vi "Init Module.vi"(8 "error in":errorcluster, 10 "Close Master Reference (F)":bool, 11 "Cloneable Module Admin in":refnum<class "Delacor_lib_QMH_Cloneable Module Admin.lvclass">) -> (0 "error out":errorcluster, 1 "Data Viewer Broadcast Events":T1, 2 "Data Viewer Request Events":T2, 3 "Cloneable Module Admin out":refnum<class "Delacor_lib_QMH_Cloneable Module Admin.lvclass">)   [LabVIEW 2020, in "Data Viewer.lvlib"]
doc: "Initialize the module by creating Broadcast Events, Request Events, and synchronization rendezvous. Also, since this is a cloneable module, add it to the cloneable registry and update the Module Admin class.\n\nSee the block diagram for an explanation of the 'Close Master Reference' parameter.\n_____\nBased on DQMH Project Template 7.0.1.1316."
uses:
  Data Viewer.lvlib
  <vilib>/Delacor/Delacor QMH/Libraries/Cloneable Module Admin_class/Delacor_lib_QMH_Cloneable Module Admin.lvclass
  C:/Program Files (x86)/National Instruments/LabVIEW 2020/vi.lib/Delacor/Delacor QMH/Libraries/Module Admin_class/Delacor_lib_QMH_Module Admin.lvclass
  Request Events--cluster.ctl
  Stop Argument--cluster.ctl
  Show Panel Argument--cluster.ctl
  Hide Panel Argument--cluster.ctl
  Show Diagram Argument--cluster.ctl
  Get Module Execution Status Argument--cluster.ctl
  Window Resize Argument--cluster.ctl
  Open File Argument--cluster.ctl
  Draw Plot Argument--cluster.ctl
  Set YScale Argument--cluster.ctl
  Update Curve Color Argument--cluster.ctl
  Show Value Argument--cluster.ctl
  <vilib>/Utility/miscctls.llb/LVPoint32TypeDef.ctl
  Menu Action Argument--cluster.ctl
  Update Filter Arguments Argument--cluster.ctl
  Filte Data Argument--cluster.ctl
  Restore Data Argument--cluster.ctl
  Cut Half Data Argument--cluster.ctl
  Select Point Argument--cluster.ctl
  Open Linear Measurement Argument--cluster.ctl
  Linear Measurement Close Argument--cluster.ctl
  Scale List Menu Action Argument--cluster.ctl
  Update Scale List Argument--cluster.ctl
  Initialize Plot List Argument--cluster.ctl
  Load Plot Argument--cluster.ctl
  Unload Plot Argument--cluster.ctl
  Show Hide Scale Argument--cluster.ctl
  Add Default Scale Argument--cluster.ctl
  Update Plot List Argument--cluster.ctl
  Add Virtual Cruve Argument--cluster.ctl
  Edit Curve Argument--cluster.ctl
  Broadcast Events--cluster.ctl
  Did Init Argument--cluster.ctl
  Status Updated Argument--cluster.ctl
  Error Reported Argument--cluster.ctl
  Linear Measurement Panel Closed Argument--cluster.ctl
  <vilib>/Delacor/Delacor QMH/Libraries/Module Admin_class/Delacor_lib_QMH_Module Admin.lvclass/Delacor_lib_QMH_Module Admin.ctl
  <vilib>/Delacor/Delacor QMH/Libraries/Cloneable Module Admin_class/Delacor_lib_QMH_Cloneable Module Admin.lvclass/Delacor_lib_QMH_Cloneable Module Admin.ctl
  <vilib>/Delacor/Delacor QMH/Libraries/Module Admin_class/Delacor_lib_QMH_Get External Launch.vi
  <vilib>/Delacor/Delacor QMH/Libraries/Cloneable Module Admin_class/Delacor_lib_QMH_Get Module ID.vi
  <vilib>/Delacor/Delacor QMH/Libraries/Cloneable Module Admin_class/Delacor_lib_QMH_Set Close Master Reference.vi
  <vilib>/Delacor/Delacor QMH/Libraries/Cloneable Module Admin_class/Delacor_lib_QMH_Set First.vi
  Clone Registration/Clone Registration.lvlib
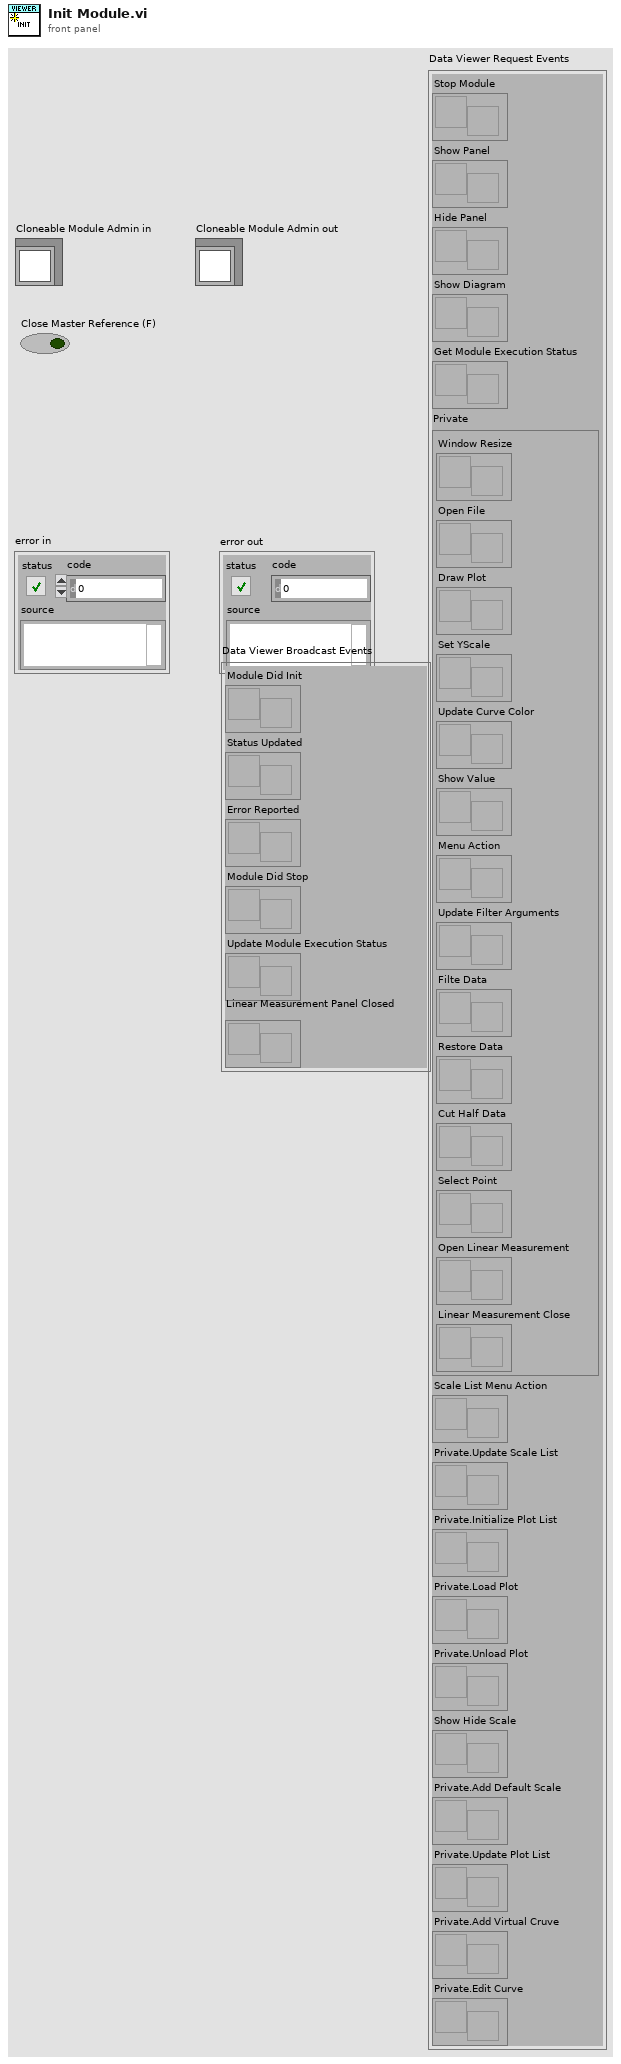
[diagram p1: front panel]
types:
  T1 = typedef "Data Viewer.lvlib/Broadcast Events--cluster.ctl" = cluster{"Module Did Init":refnum<user-event>, "Status Updated":refnum<user-event>, "Error Reported":refnum<user-event>, "Module Did Stop":refnum<user-event>, "Update Module Execution Status":refnum<user-event>, "Linear Measurement Panel Closed":refnum<user-event>}
  T2 = typedef "Data Viewer.lvlib/Request Events--cluster.ctl" = cluster{"Stop Module":refnum<user-event>, "Show Panel":refnum<user-event>, "Hide Panel":refnum<user-event>, "Show Diagram":refnum<user-event>, "Get Module Execution Status":refnum<user-event>, "Private":cluster{"Window Resize":refnum<user-event>, "Open File":refnum<user-event>, "Draw Plot":refnum<user-event>, "Set YScale":refnum<user-event>, "Update Curve Color":refnum<user-event>, "Show Value":refnum<user-event>, "Menu Action":refnum<user-event>, "Update Filter Arguments":refnum<user-event>, "Filte Data":refnum<user-event>, "Restore Data":refnum<user-event>, "Cut Half Data":refnum<user-event>, "Select Point":refnum<user-event>, "Open Linear Measurement":refnum<user-event>, "Linear Measurement Close":refnum<user-event>}, "Scale List Menu Action":refnum<user-event>, "Private.Update Scale List":refnum<user-event>, "Private.Initialize Plot List":refnum<user-event>, "Private.Load Plot":refnum<user-event>, "Private.Unload Plot":refnum<user-event>, "Show Hide Scale":refnum<user-event>, "Private.Add Default Scale":refnum<user-event>, "Private.Update Plot List":refnum<user-event>, "Private.Add Virtual Cruve":refnum<user-event>, "Private.Edit Curve":refnum<user-event>}
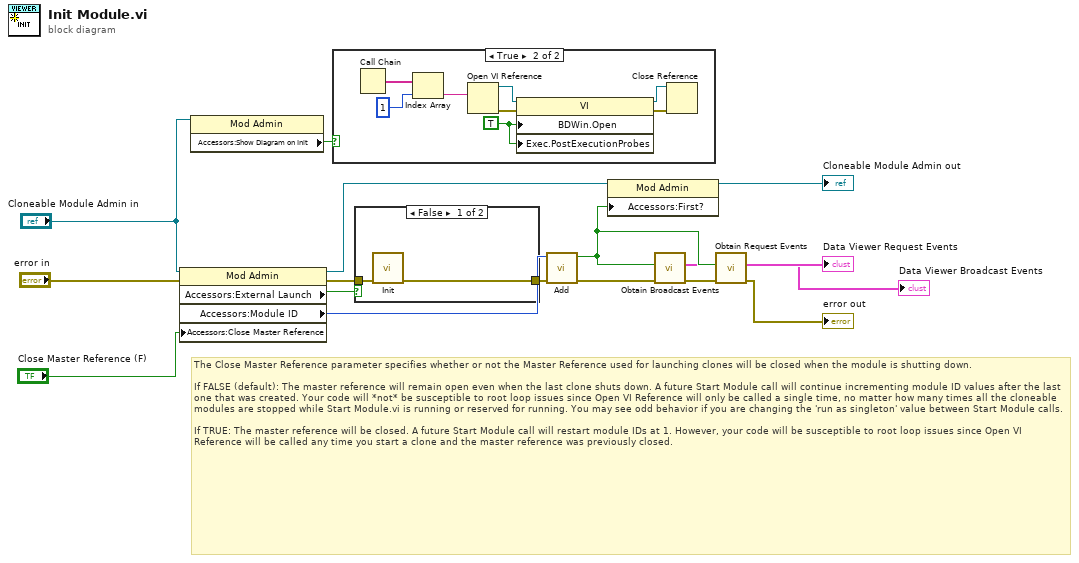
[diagram p0: block diagram]
diagram:
  # "The Close Master Reference parameter specifies whether or not the Master Reference used for launching clones will be closed when the module is shutting down. \n\nIf FALSE (default): The master reference will remain open even when the last clone shuts down. A future Start Module call will continue incrementing module ID values after the last one that was created. Your code will *not* be susceptible to root loop issues since Open VI Reference will only be called a single time, no matter how many times all the cloneable modules are stopped while Start Module.vi is running or reserved for running. You may see odd behavior if you are changing the 'run as singleton' value between Start Module calls.\n\nIf TRUE: The master reference will be closed. A future Start Module call will restart module IDs at 1. However, your code will be susceptible to root loop issues since Open VI Reference will be called any time you start a clone and the master reference was previously closed."
  n1 = property class="Mod Admin"(reference="Cloneable Module Admin in", error in="error in", "Accessors:Close Master Reference"="Close Master Reference (F)") -> (reference out=w10:refnum<class "Delacor_lib_QMH_Cloneable Module Admin.lvclass">, error out=w6:errorcluster, "Accessors:External Launch"=w9:bool, "Accessors:Module ID"=w5:i32)
  n2 = property class="Mod Admin"(reference="Cloneable Module Admin in") -> ("Accessors:Show Diagram on Init"=w3:bool)  [unwired: 1 in, 2 out]
  n3 = case shown="True" w3 {
    frame False {
    }
    frame True {
      w20 = TRUE ("Block Diagram Window:Open")
      n4 = Call Chain() -> (call chain=w24:string[])
      n5 = Index Array(array=w24, index=1) -> (element=w17:string)
      n6 = Open VI Reference(vi path=w17) -> (vi reference=w21:refnum<vi>, error out=w22:errorcluster)  [unwired: 5 in]
      n7 = property class="VI"(reference=w21, error in=w22, "BDWin.Open"=w20, "Exec.PostExecutionProbes"=w20) -> (reference out=w18:refnum<vi>, error out=w19:errorcluster)
      n8 = Close Reference(reference=w18, error in (no error)=w19) -> ()  [unwired: 1 out]
    }
  }
  n9 = case "External Launch?" shown="False" w9 {
    tunnel: [w26 w27] -> w15
    tunnel: w6 -> [w25 w27]
    frame False {
      n10 = call "Init.vi"("error in"=w25) -> ("error out"=w26:errorcluster)  [unwired: 7 in, 3 out]
    }
    frame True {
      # "Init of Clone's registration\nhappened at Start Module.vi"
    }
  }
  n11 = call "Add.vi"("error in"=w15, "Module ID"=w5) -> ("error out"=w16:errorcluster, "First?"=w11:bool)  [unwired: 7 in, 1 out]
  n12 = property class="Mod Admin"(reference=w10, "Accessors:First?"=w11) -> (reference out=→"Cloneable Module Admin out":refnum<class "Delacor_lib_QMH_Cloneable Module Admin.lvclass">)  [unwired: 1 in, 1 out]
  n13 = call "Obtain Broadcast Events.vi"("error in"=w16, "Create New? (F)"=w11) -> ("error out"=w14:errorcluster, "Data Viewer Broadcast Events"=→"Data Viewer Broadcast Events":T1)  [unwired: 8 in]
  n14 = call "Obtain Request Events.vi"("error in"=w14, "Create New? (F)"=w11) -> ("error out"=→"error out":errorcluster, "Data Viewer Request Events"=→"Data Viewer Request Events":T2)  [unwired: 8 in]
